vi "使用局部变量改变控制控件的值.vi"() -> ()   [LabVIEW 2021]
doc: "本VI是为《我和LabVIEW》一书编写的示例。\n关于本书的介绍请参考网页：\nhttp://ruanqizhen.spaces.live.com/blog/cns!5852D4F797C53FB6!4310.entry"
panel:
  in  "Stop":bool
  in  "input":string
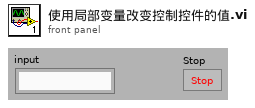
[diagram p1: front panel]
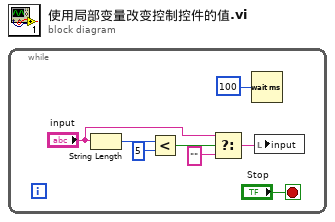
[diagram p0: block diagram]
diagram:
  n1 = while {
    stop <- "Stop" stop-if-true
    n2 = String Length(string="input") -> (length=w2:i32)
    n3 = Less?(x=w2, y=5) -> (x < y?=w7:bool)
    n4 = Select(t="input", s=w7, f="" ("字符串")) -> (s? t:f=w6:string)
    n5 = Wait (ms)(milliseconds to wait=u32 100 ("等待时间（毫秒）")) -> ()  [unwired: 1 out]
    n6 = local write "input"(w6) -> ()
  }
